vi "PosCtrl_Config_Threshold.vi"(0 "Kd":dbl, 1 "FilterDerivative":bool, 4 "Negate Output":bool, 5 "Max Allowd Position":dbl=9e+30, 6 "At Reference Count":i32=13, 7 "Min Allowd Position":dbl=-9e+30, 8 "Output Deadband":dbl=0.05, 9 "Output Threshold":dbl=1.0, 10 "ErrorDeadband":dbl=0.08, 11 "ErrorThreshold":dbl=6.0) -> (2 "Kp":dbl, 3 "PosCtrl_Config_Params":T1={"Slope"=0.0, "Offset"=0.0, "Error Deadband"=0.0, "At Reference Count"=13, "Negate Output"=FALSE, "Max Allowd Position"=9e+30, "Min Allowd Position"=-9e+30, "Kd"=0.0, "FilterDerivative"=FALSE})   [LabVIEW 2019, in "Trajectory_Library.lvlib"]
doc: "This VI creates the configuraation parameters for the position control controller. The straight line slope and intercept are calculated from the error threshold, error deadband, output threshold, and output deadband. A separate maximum output input to the controller executable allows the rate of output reduction to be constant for different maximum output values. There is also an optional Kd constant to allow a non-zero derivative term. \n\nThis position controller is really a PD controller, where Kp is the calculated slope, and Kd is specified directly, with the addition of an error deadband to compensate for sensor noise and an output deadband to compensate for static friction.\n\nThe optional inputs Max Allowed Position and Min Allowed Position provide a virtual limit switch capability that forces the output to zero when it would cause movement in the direction of the exceeded limit.\n\nThe optional \"at refernce count\" parameter specifies the number of consecutive execution cycles the absolute value of the error has to be within the deadband to set \"At Reference\" to true. For a 20 millisecond loop time, the default value of 13 forces the error to be within the deadband for 260 milliseconds before At Reference is set to true.\n\nThe optional Negate Output parameter causes the output value to be multiplied by negative one.\n\nInputs:\n - Max Allowed Position - double - (Optional,, default: 9E+30 ) \n - Max Allowed Position - double - (Optional,, default: 9E+30 ) \n - Error threshold- double - When the error reaches this point, the output will start reducing from Output Threshold to Output Deadband as the error decreases. Thie value must be positive.\n - Error Deadband - double - When the absolute value of the error is less than this, the output will be set to zero. Thie value must be positive.\n - Output Threshold - double - This is the output value used to calculate the slope of the slow down. The actual Maximum Output is specified in the Execute VI. The actual Maximum output can be greater or smaller than this value. Thie value must be positive.\n - Output Deadband - double - This is the output value when error reaches the Error Deadband. Thie value must be positive.\n - At Reference count - integer - The number of consecutive cycles that the error has to be within the Error Deadband to set the At Reference output to TRUE. (Optional, default: 13 )\n - Negate Output - boolean - When TRUE causes the output to be negated. (Optional, default: FALSE)\n - Kd - double - Derivative constant. Amount to multiply by the derivative of the Error. (Default: 0)\n\nOutputs:\n - PosCtrl_Config_Params - cluster - Data cluster containing the configuration parameters for the Position Control Execute VI.\n - Kp - double - The calculated slope, or Kp of this controller.\n - FilterDerivative - boolean - When TRUE the derivative term will be filtered by averaging the last 3 values (Default: False)"
uses:
  Trajectory_Library.lvlib
  TypeDef/PosCtrl_Tuning_Type.ctl
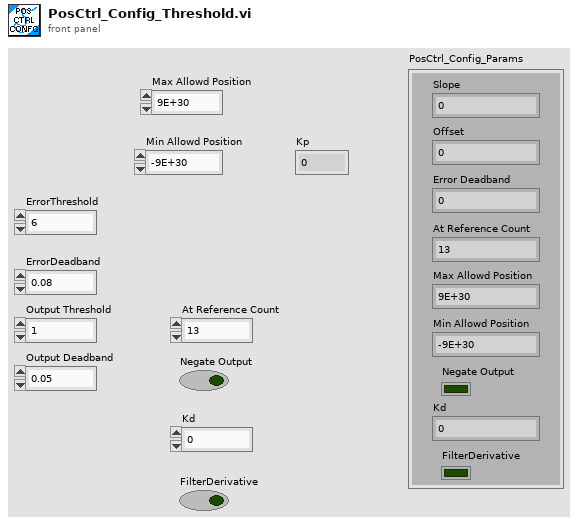
[diagram p1: front panel]
types:
  T1 = typedef "Trajectory_Library.lvlib/PosCtrl_Tuning_Type.ctl" = cluster{"Slope":dbl, "Offset":dbl, "Error Deadband":dbl, "At Reference Count":i32, "Negate Output":bool, "Max Allowd Position":dbl, "Min Allowd Position":dbl, "Kd":dbl, "FilterDerivative":bool}
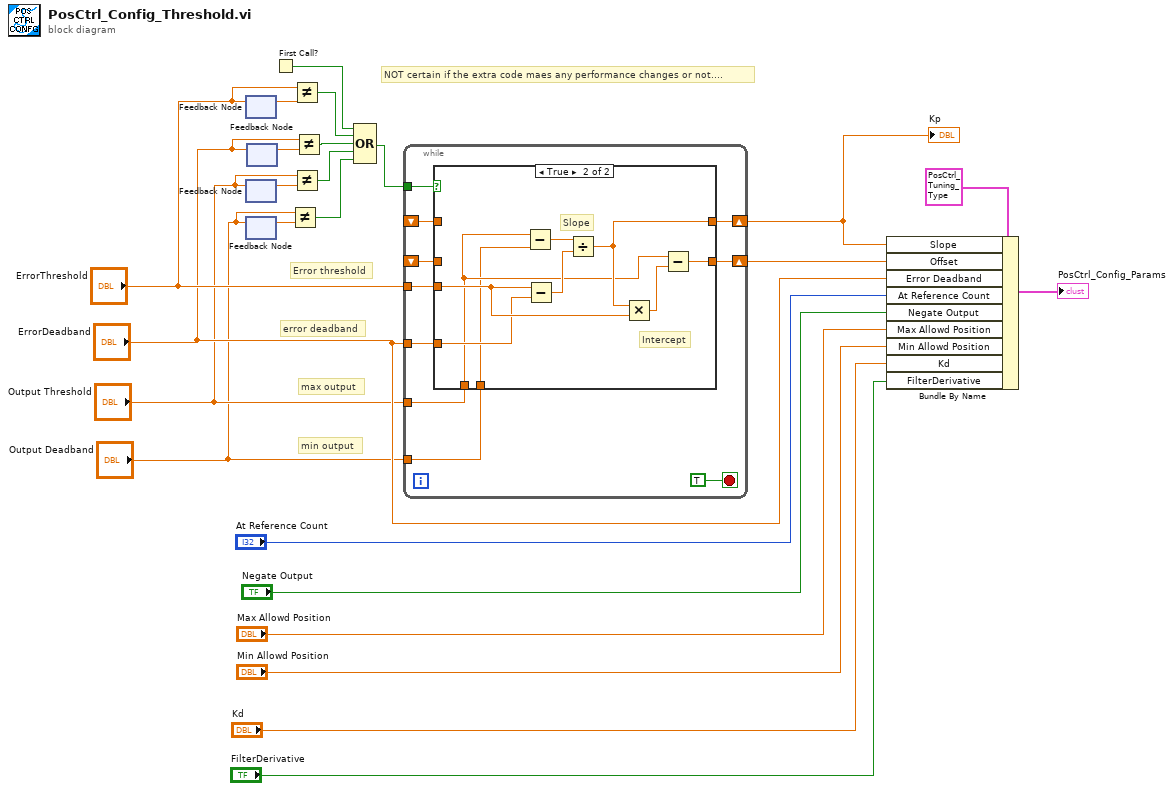
[diagram p0: block diagram]
diagram:
  # "NOT certain if the extra code maes any performance changes or not...."
  # "min output"
  # "Error threshold"
  # "error deadband"
  # "max output"
  n1 = feedback-in #1("ErrorThreshold") -> ()
  n2 = feedback #1() -> (w16:dbl)  [unwired: 1 in]
  n3 = feedback #2() -> (w12:dbl)  [unwired: 1 in]
  n4 = feedback-in #2("Output Threshold") -> ()
  n5 = feedback #3() -> (w10:dbl)  [unwired: 1 in]
  n6 = feedback-in #3("Output Deadband") -> ()
  n7 = feedback #4() -> (w14:dbl)  [unwired: 1 in]
  n8 = feedback-in #4("ErrorDeadband") -> ()
  n9 = First Call?() -> (First Call?: T/F=w4:bool)
  n10 = Not Equal?(x="Output Deadband", y=w10) -> (x != y?=w5:bool)
  n11 = Not Equal?(x="ErrorThreshold", y=w16) -> (x != y?=w8:bool)
  n12 = Not Equal?(x="Output Threshold", y=w12) -> (x != y?=w6:bool)
  n13 = Not Equal?(x="ErrorDeadband", y=w14) -> (x != y?=w7:bool)
  n14 = Compound Arithmetic op=OR(w4, w8, w7, w6, w5) -> (w3:bool)
  n15 = while {
    tunnel: "ErrorThreshold" -> [w32]
    tunnel: "ErrorDeadband" -> [w31]
    tunnel: "Output Threshold" -> [w30]
    tunnel: "Output Deadband" -> [w29]
    tunnel: w3 -> [w28]
    shift-right: [w34] -> w22
    shift-left: _ -> [w27]
    shift-right: [w33] -> w21
    shift-left: _ -> [w26]
    stop <- TRUE stop-if-true
    n16 = case shown="True" w28 {
      tunnel: [w36 w42] -> w34
      tunnel: [w35 w41] -> w33
      tunnel: w32 -> [_ w40]
      tunnel: w31 -> [_ w39]
      tunnel: w30 -> [_ w38]
      tunnel: w29 -> [_ w37]
      tunnel: w27 -> [w36 _]
      tunnel: w26 -> [w35 _]
      frame False {
      }
      frame True {
        # "Slope"
        # "Intercept"
        n17 = Subtract(x=w38, y=w37) -> (x-y=w43:dbl)
        n18 = Subtract(x=w40, y=w39) -> (x-y=w44:dbl)
        n19 = Divide(x=w43, y=w44) -> (x/y=w42:dbl)
        n20 = Multiply(x=w42, y=w40) -> (x*y=w45:dbl)
        n21 = Subtract(x=w38, y=w45) -> (x-y=w41:dbl)
      }
    }
  }
  "Kp" <- w22
  n22 = Bundle By Name(cluster=T1 {"Slope"=0.0, "Offset"=0.0, "Error Deadband"=0.0, "At Reference Count"=13, "Negate Output"=FALSE, "Max Allowd Position"=9e+30, "Min Allowd Position"=-9e+30, "Kd"=0.0, "FilterDerivative"=FALSE} ("PosCtrl_Config_Params"), "Slope"=w22, "Offset"=w21, "Error Deadband"="ErrorDeadband", "At Reference Count"="At Reference Count", "Negate Output"="Negate Output", "Max Allowd Position"="Max Allowd Position", "Min Allowd Position"="Min Allowd Position", "Kd"="Kd", "FilterDerivative"="FilterDerivative") -> (→"PosCtrl_Config_Params":T1)
